vi "Variable glob Edwards.vi"() -> ()   [LabVIEW 2022 SP3]
uses:
  Pressions/Gestion grappe/TypeDef_Seuil Jauge Pression_CN.ctl
panel:
  in  "Seuil Jauge":T1={"Descente en Pression"={"Min Mesure Piezo"=5.0, "Min Mesure Pirani"=0.0002}, "Montée en Pression"={"Max Mesure Pirani"=10.0, "Max Mesure Penning"=0.0004}} {"Montée en Pression"."Max Mesure Penning" format="%.2e"; "Montée en Pression"."Max Mesure Pirani" format="%.2e"; "Descente en Pression"."Min Mesure Pirani" format="%.2e"; "Descente en Pression"."Min Mesure Piezo" format="%.2e"}
  out "Donnees pour grappes":dbl[][](array[numeric])
  in  "Donnees Grappes":string[](array[string])
  in  "Nom select grappes":string[](array[string])
  in  "Select Grappes":bool[](array[boolean])
  out "Grappes":string[][](array[string])
  in  "Refnum Edwards":refnum<vi>
  in  "Donnees Edwards 1D":string[](array[string])
  in  "Nom select Edwards":string[](array[string])
  in  "Donnees Edwards":string[][](array[string])
  in  "Select Edwards":bool[][](array[boolean])
  in  "Noms Edwards":string[][](array[string])
  in  "Voies Pres Edwards":i8[][](array[numeric])
  in  "EDWARDS":bool
  in  "Port RS232 Edwards":refnum<visa-resource-name>[](array[refnum])
  # "Donnees (pour les tableaux 2D, colonnes = differents TIC)"
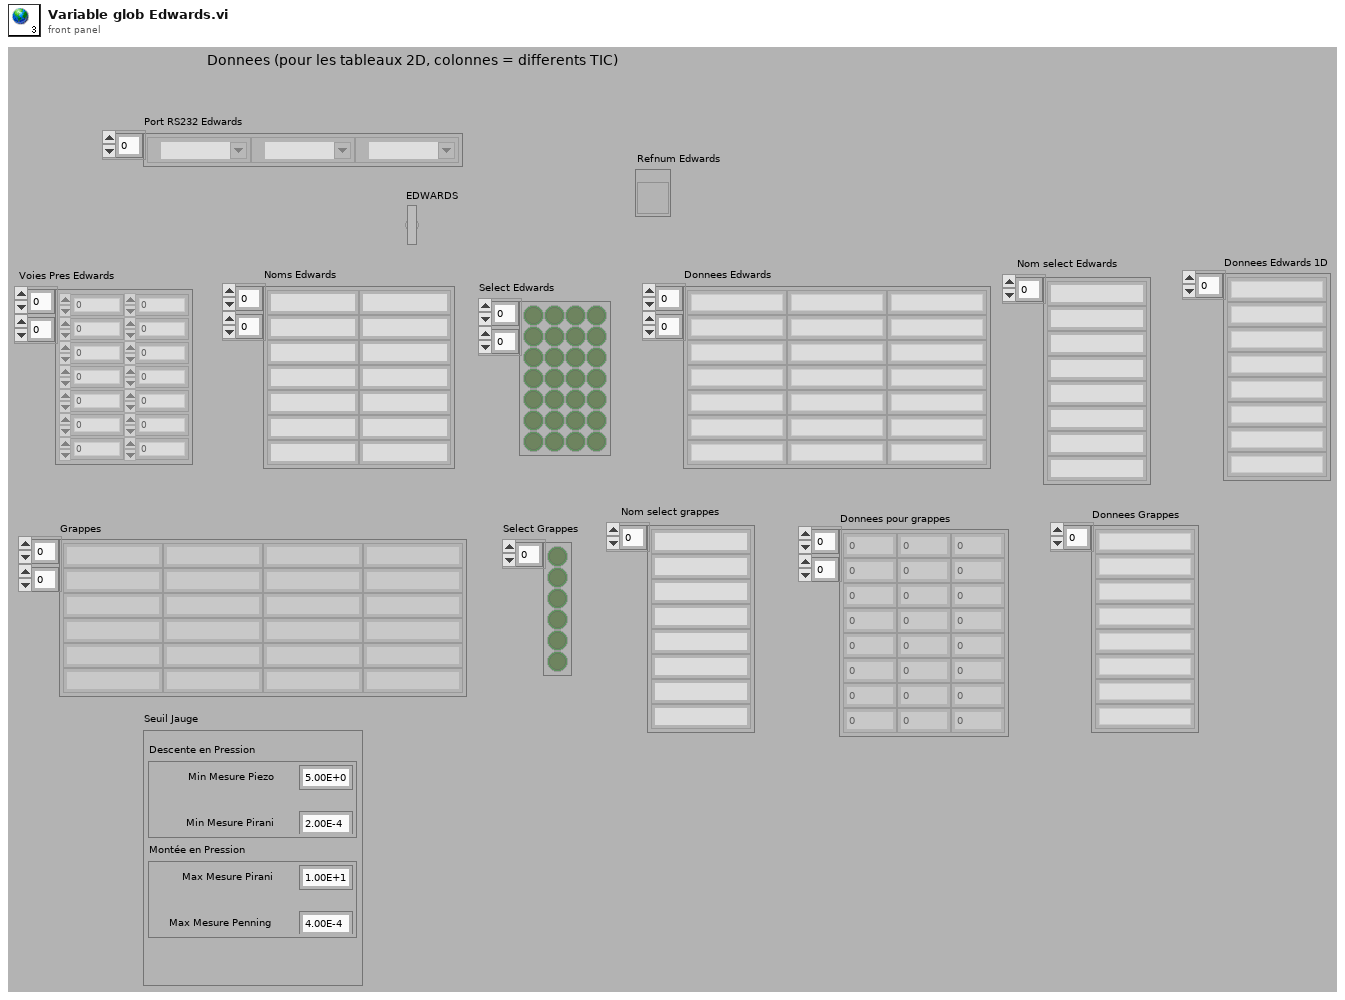
[diagram p1: front panel]
types:
  T1 = typedef "TypeDef_Seuil Jauge Pression_CN.ctl" = cluster{"Descente en Pression":cluster{"Min Mesure Piezo":dbl, "Min Mesure Pirani":dbl}, "Montée en Pression":cluster{"Max Mesure Pirani":dbl, "Max Mesure Penning":dbl}}
diagram:
